vi "from string array.vi"(8 "error in (no error)":errorcluster, 9 "String Array":string[][](array[string]), 10 "version":string, 11 "module configuration in":refnum<class "Modbus Module configuration.lvclass">) -> (0 "error out":errorcluster, 3 "module configuration out":refnum<class "Modbus Module configuration.lvclass">)   [LabVIEW 2015, in "Modbus Module configuration.lvclass"]
uses:
  Modbus Module configuration.lvclass
  module channel/Modbus Module Channel.lvclass
  <vilib>/NI/Tag Bus/tag/Data Type.ctl
  editor node/permissions.ctl
  <vilib>/NI/Tag Bus/tag/tag descriptor.lvclass/tag descriptor.ctl
  <vilib>/NI/Tag Bus Module Framework/channel/TBM channel.lvclass/TBM channel.ctl
  Modbus Module configuration.lvclass/Modbus Module configuration.ctl
  <vilib>/NI/Tag Bus/tag/tag descriptor.lvclass
  editor node/Modbus Module editor node.lvclass
  <vilib>/NI/Tag Bus Module Framework/channel/TBM channel.lvclass
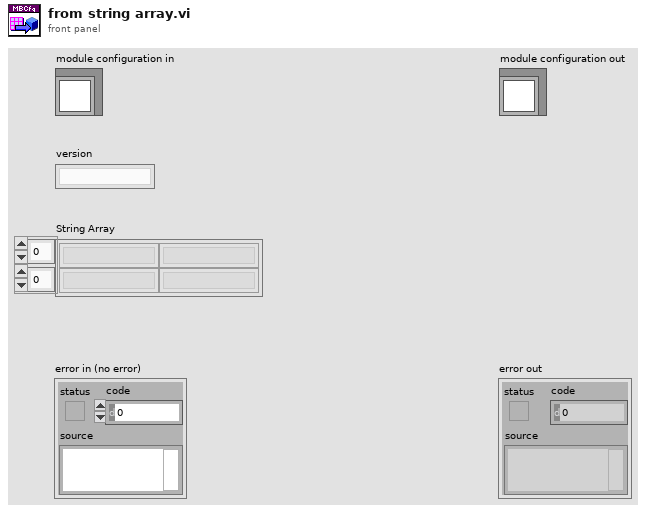
[diagram p1: front panel]
types:
  T1 = typedef "Modbus Module editor node.lvclass/permissions.ctl" = enum32{"Read from MB", "Write to MB"}
  T2 = typedef "tag bus.lvlib/tag descriptor.lvclass/Data Type.ctl" = enum16{"Double", "Single", "I64", "I32", "I16", "I8", "U64", "U32", "U16", "U8", "Boolean", "String", "Array of Double", "Array of Single", "Array of I64", "Array of I32", "Array of I16", "Array of I8", "Array of U64", "Array of U32", "Array of U16", "Array of U8", "Array of Boolean", "Array of String"}
  T3 = typedef "TBM channel.lvclass/channel classification.ctl" = enum16{"input data", "output data", "processing parameter", "processing result"}
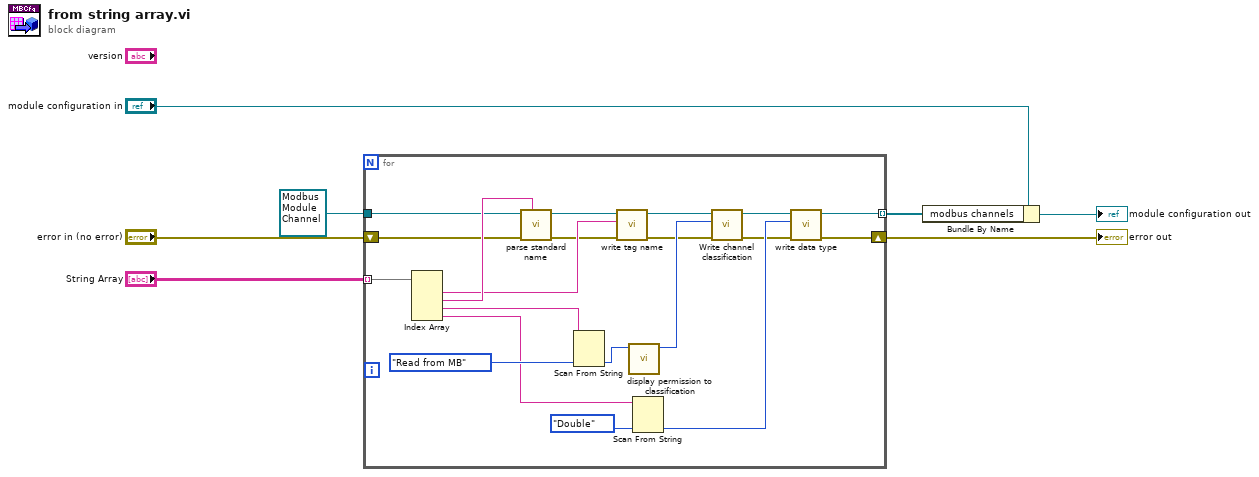
[diagram p0: block diagram]
diagram:
  n1 = for {
    tunnel: "String Array" -> [w27] mode=indexing
    tunnel: refnum<class "Modbus Module Channel.lvclass"> refnum ("Modbus Module Channel in") -> [w20]
    tunnel: [w14] -> w3 mode=indexing
    shift-right: [w8] -> w1
    shift-left: "error in (no error)" -> [w12]
    n2 = Index Array(array=w27) -> (element #1=w18:string, element #2=w21:string, element #3=w25:string, element #4=w22:string)  [unwired: 4 in]
    n3 = call "parse standard name.vi"("standard name"=w21, "error in"=w12, "Modbus Module Channel in"=w20) -> ("error out"=w11:errorcluster, "Modbus Module Channel out"=w19:refnum<class "Modbus Module Channel.lvclass">)  [unwired: 7 in]
    n4 = Scan From String(input string=w25, default 1=permissions."Read from MB" ("permissions")) -> (output 1=w23:T1)  [unwired: 3 in, 3 out]
    n5 = call <vilib>:"write tag name.vi"("error in"=w11, "name"=w18, "system tag in"=w19) -> ("error out"=w10:errorcluster, "system tag out"=w17:refnum<class "Modbus Module Channel.lvclass">)  [unwired: 7 in]
    n6 = call "display permission to classification.vi"("display permissions"=w23) -> ("channel classification"=w16:T3)  [unwired: 10 in]
    n7 = Scan From String(input string=w22, default 1=Data_Type."Double" ("data type")) -> (output 1=w13:T2)  [unwired: 3 in, 3 out]
    n8 = call <vilib>:"Write channel classification.vi"("error in"=w10, "channel classification"=w16, "channel in"=w17) -> ("error out"=w9:errorcluster, "channel out"=w15:refnum<class "Modbus Module Channel.lvclass">)  [unwired: 7 in]
    n9 = call <vilib>:"write data type.vi"("error in"=w9, "data type"=w13, "system tag in"=w15) -> ("error out"=w8:errorcluster, "system tag out"=w14:refnum<class "Modbus Module Channel.lvclass">)  [unwired: 7 in]
  }
  "error out" <- w1
  n10 = Bundle By Name(cluster="module configuration in", "modbus channels"=w3) -> (→"module configuration out":refnum<class "Modbus Module configuration.lvclass">)
